vi "[ex ce] CSE - VI control and data exchange.vi"() -> ()   [LabVIEW 2021]
doc: "This is example of using CalcExpress Script Engine (CSE).\n\nThe example demonstrates how you can control VIs in a CSE script. Also, it shows various methods that can be used to exchange data between scripts and VIs.\n\n::: CalcExpress Toolkit :::\nCopyright (c) 2000-2026 Konstantin Shifershteyn. All rights reserved."
panel:
  out "graph":dbl[][](graph)
  in  "finished":bool
  in  "stop":bool
  in  "Script":string="viName = \"Exmpl - Signal Generator.vi\";             /* name of VI to run */\nviPath = FileBuildPath(FileGetAppPath(1), viName);  /* VI full path */\n\n/* Test if the Signal Generator VI is already running */\nif (viState(viName) < 2) {\n  /* If the VI is not running */\n  /* Assigns values to VI's controls and runs the VI */\n  viRun(viPath, 1, \"samples\",512, \"noise amplitude\",1.5);\n  if (lvErrorMessage(\"viRun function\"))\n    return -1;                     /* exit if error */\n}\nelse {\n  /* If the VI is already running */\n  /* Assigns values to VI's controls */\n  viCtrlSet(viName, \"samples\",512, \"noise amplitude\",1.5);\n  if (lvErrorMessage(\"viCtrlSet function\"))\n    return -1;                     /* exit if error */\n}\n\n/* Obtain a Notifier name from the control on the VI's Front Panel */\nnotif = \"\";                        /* declare a variable for Notifier name */\nviCtrlGet(viName, \"Notifier\", notif);\nif (lvErrorMessage(\"viCtrlGet function\"))\n  return -2;\n\nviCtrlSet(viName, \"generate\",1);   /* forces the VI to generate data */\n\n/* Do while the Generator VI is running */\nwhile(viState(viName) > 1) {\n\n   msg = NotifWait(notif,100,0);   /* wait for a notification */\n   if (errno() == 56)              /* repeat if time-out */\n      continue;\n   if (lvErrorMessage(\"NotifWait function\"))\n      return -4;                   /* exit if an error */\n\n   if (!sccmp(msg, \"Halt\"))        /* exit if halt notification */\n      return 0;\n\n   /* parsing a notification */\n   src = smatch(msg,\"=\",-1);\n   nam = smatch(msg,\"=\",1);\n   probe(vector(msg,src,nam), \"Notification\",0,0);   /*display*/\n\n   if (!sccmp(src, \"Data:fpControl\")) {\n      /* get data directly from the specified FP indicator */\n      viCtrlGet(viName, nam, data);\n   }\n   else if (!sccmp(src, \"Data:File\")) {\n      /* read data from the specified file */\n      FileLoadSS(nam, data, 1);\n   }\n   else if (!sccmp(src, \"Data:Queue\")) {\n      /* get data from the specified queue */\n      data = ss2dbl(QueueGet(nam,0))[0];\n   }\n   else if (!sccmp(src, \"Data:Var\")) {\n      /* Get data from the specified variable in the specified context */\n      cntx = smatch(nam, \":\", -1);             /* context handle (string)*/\n      name = smatch(nam, \":\",  1);             /* variable name */\n      probe(vector(cntx,name), \"Context handle and variable name\");\n      err = vcopy(name, \"data\", siton(cntx));  /* copy variable */\n      if (err)\n         MsgBox(\"Error of copying variable: \", err);\n   }\n   else {\n      MsgBox(\"Unrecognized notification: \", msg);\n      continue;\n   }\n\n   /* --- data processing --- */\n   len = size(data);\n   fft = fft(data);\n   mag = norm(fft[0:len/2]);\n   pha = arg (fft[0:len/2]);\n\n   cyc = search(mag, max(mag));\n   amp = 2*max(mag)/len;\n   res = pSine(len, amp, 0, cyc);\n\n   /* signals the fact data are ready */\n   count += 1;\n}\nreturn 1;\n"
  # "This example demonstrates how you can control VIs from a script.\nAlso, it shows various methods that can be used to exchange data between scripts and VIs."
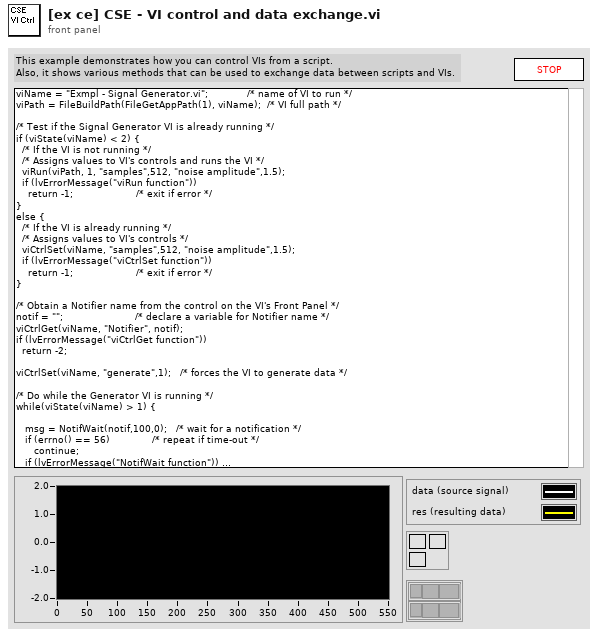
[diagram p1: front panel]
types:
  T1 = enum32{"nothing", "reset", "assign name", "get name", "get handle"}
  T2 = enum16{"create", "destroy", "set value", "get value"}
  T3 = typedef "VarMan Variable Context Handle.ctl" = i32
  T4 = typedef "CSE Instance RefNum.ctl" = refnum<k1>
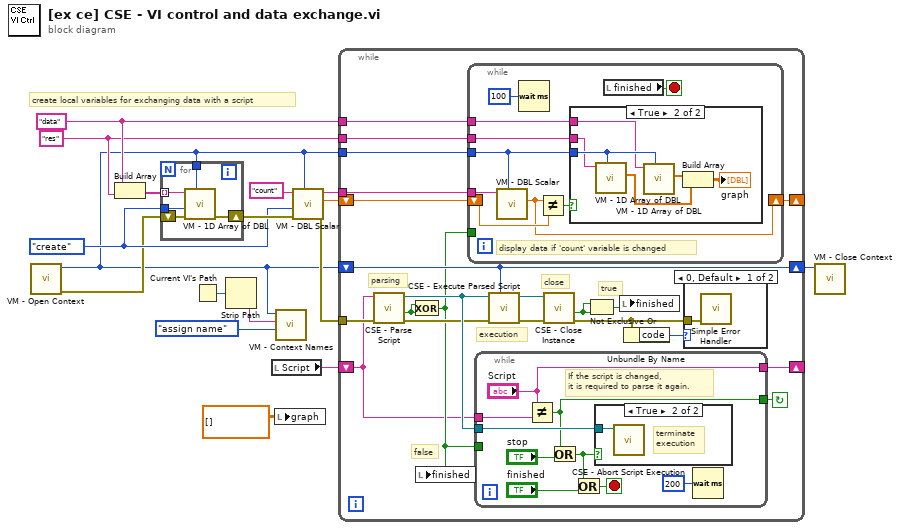
[diagram p0: block diagram]
diagram:
  w9 = "res"
  w10 = "data"
  w14 = T2."create" ("cmd")
  # "create local variables for exchanging data with a script"
  n1 = call "VM - Open Context.vi"() -> ("error out"=w13:errorcluster, "VC Handle out"=w2:T3)  [unwired: 9 in, 1 out]
  n2 = Build Array(w10, w9) -> (w11:string[])
  n3 = for {
    shift-right: [w20] -> w15
    shift-left: w13 -> [w22]
    tunnel: w11 -> [w21] mode=indexing
    tunnel: w14 -> [w19]
    tunnel: w2 -> [w18]
    n4 = call "VM - 1D Array of DBL.vi"("VC Handle"=w18, "error in"=w22, "cmd"=w19, "name_spec"=w21) -> ("error out"=w20:errorcluster)  [unwired: 2 in, 5 out]
  }
  n5 = Current VI's Path() -> (path=w3:path)
  n6 = Strip Path(path=w3) -> (name=w4:string)  [unwired: 1 out]
  n7 = local read "Script"() -> (w1:string)
  n8 = local write "graph"(dbl[][] [] ("graph")) -> ()
  n9 = call "VM - Context Names.vi"("action"=T1."assign name", "VC Name"=w4, "VC Handle"=w2) -> ()  [unwired: 3 in, 4 out]
  n10 = call "VM - DBL Scalar.vi"("VC Handle"=w2, "error in"=w15, "cmd"=w14, "name_spec"="count" ("name")) -> ("error out"=w12:errorcluster, "value out"=w16:dbl, "dup name_spec"=w8:string)  [unwired: 2 in, 3 out]
  n11 = while {
    tunnel: w8 -> [w25]
    tunnel: w9 -> [w26]
    tunnel: w10 -> [w27]
    tunnel: w2 -> [w32]
    shift-left: w16 -> [w31]
    shift-right: [w30] -> _
    tunnel: w12 -> [w33]
    shift-right: [w24] -> _
    shift-left: w1 -> [w23]
    shift-right: [w34] -> w17
    shift-left: w2 -> [w34]
    stop <- w28 continue-if-true
    # "true"
    # "false"
    # "close"
    # "execution"
    # "parsing"
    n12 = call "CSE - Parse Script.vi"("error in"=w33, "Script"=w23) -> ("error out"=w39:errorcluster, "dynamic instance"=w38:bool, "CSE RefNum"=w41:T4)  [unwired: 5 in, 2 out]
    n13 = Exclusive Or(1:w38, 2:w38) -> (0:w29:bool)
    n14 = local write "finished"(w29) -> ()
    n15 = while {
      tunnel: w26 -> [w55]
      tunnel: w27 -> [w56]
      tunnel: w29 -> [_]
      shift-left: w31 -> [w59]
      shift-right: [w58] -> w30
      tunnel: w25 -> [w62]
      tunnel: w32 -> [w60]
      stop <- w54 stop-if-true
      # "display data if 'count' variable is changed"
      n16 = call "VM - DBL Scalar.vi"("VC Handle"=w60, "name_spec"=w62) -> ("value out"=w58:dbl)  [unwired: 4 in, 5 out]
      n17 = Wait (ms)(milliseconds to wait=u32 100) -> ()  [unwired: 1 out]
      n18 = Not Equal?(x=w58, y=w59) -> (x != y?=w61:bool)
      n19 = case shown="True" w61 {
        tunnel: w60 -> [_ w68]
        tunnel: w56 -> [_ w64]
        tunnel: w55 -> [_ w63]
        frame False {
        }
        frame True {
          n20 = call "VM - 1D Array of DBL.vi"("VC Handle"=w68, "name_spec"=w63) -> ("value out"=w66:dbl[])  [unwired: 4 in, 5 out]
          n21 = call "VM - 1D Array of DBL.vi"("VC Handle"=w68, "name_spec"=w64) -> ("value out"=w67:dbl[])  [unwired: 4 in, 5 out]
          n22 = Build Array(w67, w66) -> (→"graph":dbl[][])
        }
      }
      n23 = local read "finished"() -> (w54:bool)
    }
    n24 = while {
      tunnel: [w45] -> w28
      tunnel: w23 -> [w47]
      tunnel: w29 -> [_]
      tunnel: w41 -> [w52]
      tunnel: ["Script"] -> w24
      stop <- w50 stop-if-true
      # "If the script is changed,\nit is required to parse it again."
      n25 = Not Equal?(x="Script", y=w47) -> (x != y?=w45:bool)
      n26 = Or(x=w45, y="stop") -> (x .or. y?=w46:bool)
      n27 = Or(x=w46, y="finished") -> (x .or. y?=w50:bool)
      n28 = case shown="True" w46 {
        tunnel: w52 -> [_ w53]
        frame False {
        }
        frame True {
          # "terminate\nexecution"
          n29 = call "CSE - Abort Script Execution.vi"("CSE RefNum"=w53) -> ()  [unwired: 6 in, 3 out]
        }
      }
      n30 = Wait (ms)(milliseconds to wait=u32 200) -> ()  [unwired: 1 out]
    }
    n31 = call "CSE - Execute Parsed Script.vi"("VC Handle"=w34, "error in"=w39, "CSE RefNum"=w41) -> ("error out"=w42:errorcluster, "dup CSE RefNum"=w43:T4)  [unwired: 4 in, 3 out]
    n32 = call "CSE - Close Instance.vi"("error in"=w42, "CSE RefNum"=w43) -> ("error out"=w37:errorcluster, "destroyed"=w40:bool)  [unwired: 5 in, 1 out]
    n33 = Not Exclusive Or(1:w40, 2:w40) -> (0:w35:bool)
    n34 = local write "finished"(w35) -> ()
    n35 = Unbundle By Name(w37) -> ("code"=w36:i32)
    n36 = case shown="0, Default" w36 {
      tunnel: w37 -> [w69 _]
      frame 0, Default {
        n37 = call <vilib>:"Simple Error Handler.vi"("error in (no error)"=w69) -> ()  [unwired: 4 in, 5 out]
      }
      frame 7104 {
        # "abort"
      }
    }
  }
  n38 = call "VM - Close Context.vi"("VC Handle"=w17) -> ()  [unwired: 9 in, 2 out]
